vi "insert_edge.vi"(10 "edge":refnum<class "Edge.lvclass">, 11 "digraph":refnum<class "DiGraph.lvclass">) -> (1 "edge unchanged?":bool, 2 "edge already included?":bool, 3 "digraph out":refnum<class "DiGraph.lvclass">)   [LabVIEW 2020, in "graph.lvlib" / "DiGraph.lvclass"]
uses:
  DiGraph.lvclass
  Edge/Edge.lvclass
  DiGraph.lvclass/DiGraph.ctl
  4775521a-dcdb-4985-b41c-6a23402e0cd2.vi
  192cd781-888a-4283-9972-3738ebc0cdeb.vi
  Graph/Graph.lvclass
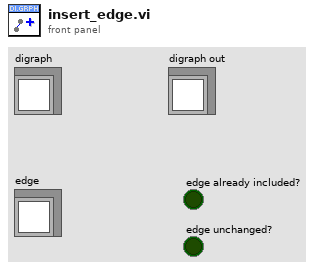
[diagram p1: front panel]
types:
  T1 = typedef "edge-definition-cluster.ctl" = cluster{"source-id":refnum<class "ID.lvclass">, "sink-id":refnum<class "ID.lvclass">}
  T2 = map{refnum<class "ID.lvclass">, set{refnum<class "ID.lvclass">}}
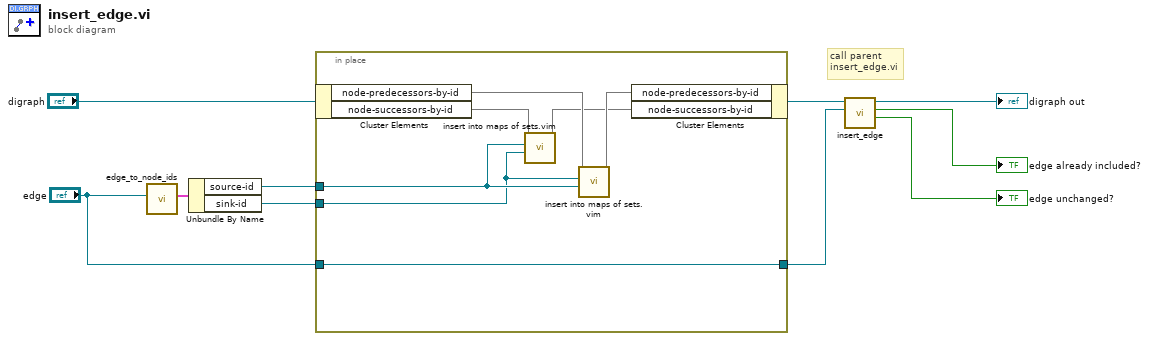
[diagram p0: block diagram]
diagram:
  # "call parent\ninsert_edge.vi"
  n1 = call "edge_to_node_ids.vi"("edge"="edge") -> ("node-ids-cluster"=w4:T1)  [unwired: 10 in]
  n2 = Unbundle By Name(w4) -> ("source-id"=w3:refnum<class "ID.lvclass">, "sink-id"=w1:refnum<class "ID.lvclass">)
  n3 = in-place {
    in-place-border: "edge" -> [w15]
    in-place-border: [w15] -> w7
    in-place-border: w3 -> [w12]
    in-place-border: w1 -> [w11]
    n4 = in-place-cluster #1("digraph") -> ("node-predecessors-by-id"=w17:T2, "node-successors-by-id"=w14:T2)
    n5 = call "insert into maps of sets.vim"("value"=w11, "key"=w12, "map of sets in"=w14) -> ("map of sets out"=w13:T2)  [unwired: 8 in]
    n6 = call "insert into maps of sets.vim"("value"=w12, "key"=w11, "map of sets in"=w17) -> ("map of sets out"=w16:T2)  [unwired: 8 in]
    n7 = in-place-cluster #1("node-predecessors-by-id"=w16, "node-successors-by-id"=w13) -> (w9:refnum<class "DiGraph.lvclass">)
  }
  n8 = call-parent "insert_edge.vi"("edge"=w7, "graph"=w9) -> ("edge unchanged?"=→"edge unchanged?":bool, "edge already included?"=→"edge already included?":bool, "graph out"=→"digraph out":refnum<class "DiGraph.lvclass">)  [unwired: 7 in]
